vi "Configure Module.vi"(8 "error in (no error)":errorcluster, 10 "IOV ref in":variant, 11 "Module Template in":refnum<class "9203.lvclass">) -> (0 "error out":errorcluster, 2 "IOV ref out":variant, 3 "Module Template out":refnum<class "9203.lvclass">)   [LabVIEW 2020, in "Modules.lvlib" / "9203.lvclass"]
uses:
  9203.lvclass
  <resource>/objmgr/cRIO.rc
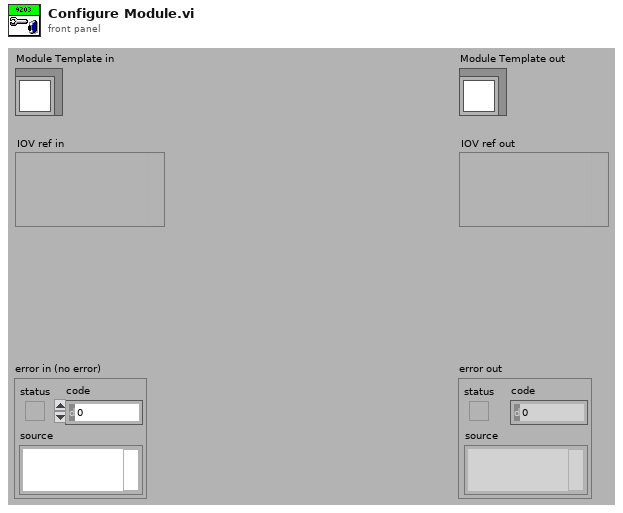
[diagram p1: front panel]
types:
  T1 = typedef "Modules.lvlib/9203.lvclass/Channel Settings.ctl" = cluster{"Range":T2}[]
  T2 = typedef "Modules.lvlib/9203.lvclass/Range.ctl" = u32
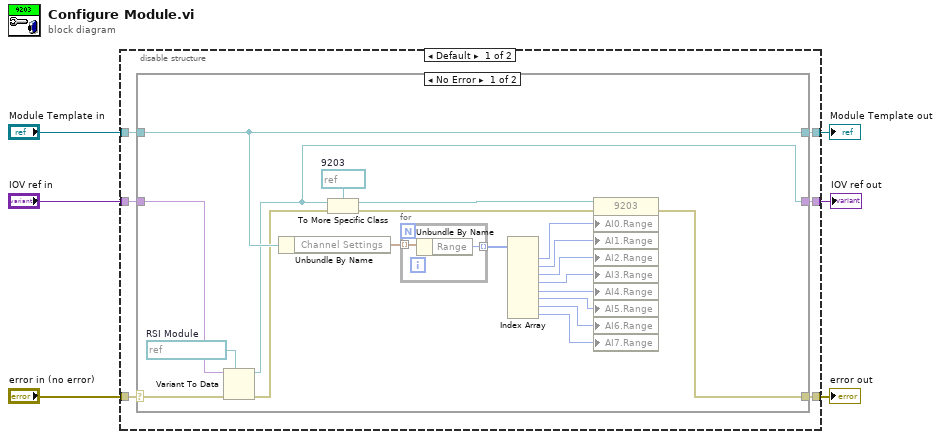
[diagram p0: block diagram]
diagram:
  n1 = disable-structure shown="Default" {
    disable-tunnel: "error in (no error)" -> [w12 w40]
    disable-tunnel: [w11 w40] -> w5
    disable-tunnel: "Module Template in" -> [w10 w38]
    disable-tunnel: [w9 w38] -> w3
    disable-tunnel: "IOV ref in" -> [w8 w39]
    disable-tunnel: [w7 w39] -> w1
    frame condition #0 {
      n2 = case shown="No Error" w12 {
        selector: w12 -> [w17 w37]
        tunnel: [w28 w37] -> w11
        tunnel: [w32 w36] -> w9
        tunnel: w10 -> [w32 w36]
        tunnel: w8 -> [w15 w35]
        tunnel: [w14 w35] -> w7
        frame No Error {
          w13 = refnum<k21> refnum  # RSI Module
          w31 = refnum<k21> refnum  # 9203
          n3 = Variant To Data(error in=w17, type=w13, Variant=w15) -> (data=w14:refnum<k21>, error out=w16:errorcluster)
          n4 = Unbundle By Name(w32) -> ("Channel Settings"=w27:T1)
          n5 = To More Specific Class(target class=w31, reference=w14, error in=w16) -> (specific class reference=w30:refnum<k21>, error out=w29:errorcluster)
          n6 = for {
            tunnel: w27 -> [w34] mode=indexing
            tunnel: [w33] -> w26 mode=indexing
            n7 = Unbundle By Name(w34) -> ("Range"=w33:T2)
          }
          n8 = Index Array(array=w26) -> (element #1=w25:T2, element #2=w24:T2, element #3=w23:T2, element #4=w22:T2, element #5=w21:T2, element #6=w20:T2, element #7=w19:T2, element #8=w18:T2)  [unwired: 8 in]
          n9 = property class="9203"(reference=w30, error in=w29, "AI0.Range"=w25, "AI1.Range"=w24, "AI2.Range"=w23, "AI3.Range"=w22, "AI4.Range"=w21, "AI5.Range"=w20, "AI6.Range"=w19, "AI7.Range"=w18) -> (error out=w28:errorcluster)  [unwired: 1 out]
        }
        frame Error {
        }
      }
    }
    frame condition #1 (active) {
    }
  }
  "error out" <- w5
  "Module Template out" <- w3
  "IOV ref out" <- w1
